vi "Base Level Estimation.vi"(7 "Base N info":T1, 8 "error in":errorcluster caption="エラー入力（エラーなし）", 9 "Filename":string, 10 "BR BL and STD info":T2, 11 "Raw data":dbl[](array[numeric])) -> (0 "error out":errorcluster caption="エラー出力", 2 "Data Estimated Info":T3, 3 "Relative G Data Array":dbl[](array[numeric]), 5 "Histogram Graph":T4(graph) caption="ヒストグラムグラフ")   [LabVIEW 2018]
uses:
  <vilib>/Analysis/baseanly.llb/Multimode.vi
  <vilib>/Analysis/baseanly.llb/Mean (DBL).vi
  <vilib>/Analysis/NI_AALBase.lvlib
panel:
  out "Region BL [pA]":dbl
  out "B BL [pA]":dbl
  out "H MIN Mode":dbl
  out "G level intensity":dbl
  out "要素":string
  out "Base S level":dbl[](array[numeric])
  out "Base Composition":string[](array[string])
  out "R Cut# 2":i32=15
  out "BL Level 2":dbl
  out "Mx Level intensity":dbl
  out "Mx level":dbl
  out "Histogram bin":dbl
  out "Data point":i32
  out "R Cut#":i32=15
  out "BL Level":dbl
  out "MIN":dbl
  out "MAX":dbl
  # "BL selection"
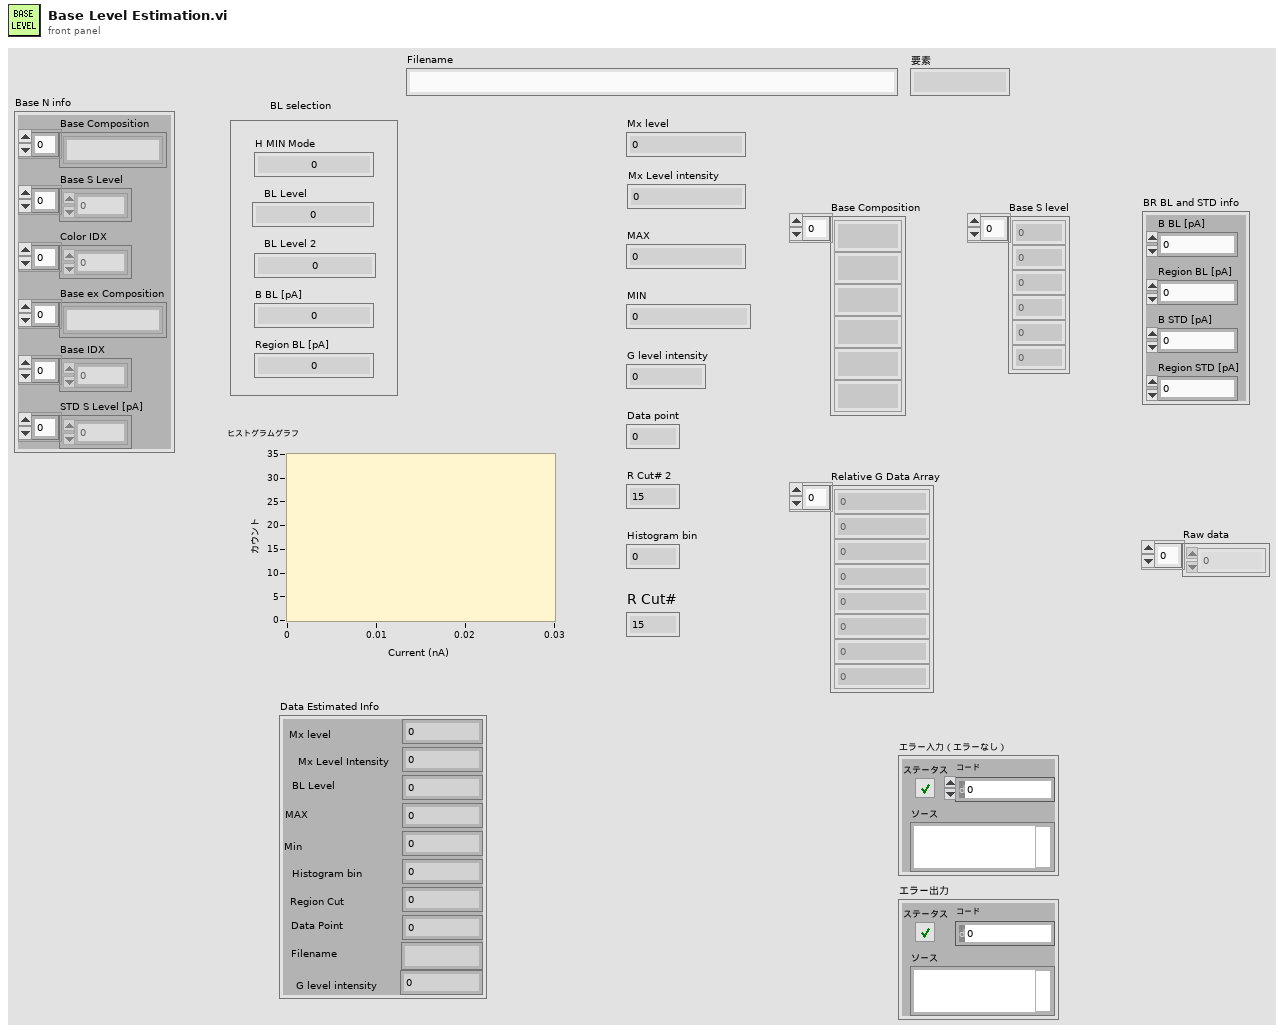
[diagram p1: front panel]
types:
  T1 = cluster{"Base Composition":string[], "Base S Level":dbl[], "Color IDX":u32[], "Base ex Composition":string[], "Base IDX":i32[], "STD S Level [pA]":dbl[]}
  T2 = cluster{"B BL [pA]":dbl, "Region BL [pA]":dbl, "B STD [pA]":dbl, "Region STD [pA]":dbl}
  T3 = cluster{"Mx level":dbl, "Mx Level Intensity":dbl, "BL Level":dbl, "MAX":dbl, "Min":dbl, "Histogram bin":dbl, "Region Cut":dbl, "Data Point":i32, "Filename":string, "G level intensity":dbl}
  T4 = cluster{"X Values":dbl[], "Histogram: h(x)":i32[]}
  T5 = cluster{dbl, dbl, dbl, dbl, dbl, "上限":dbl, dbl, i32, "Filename":string, dbl}
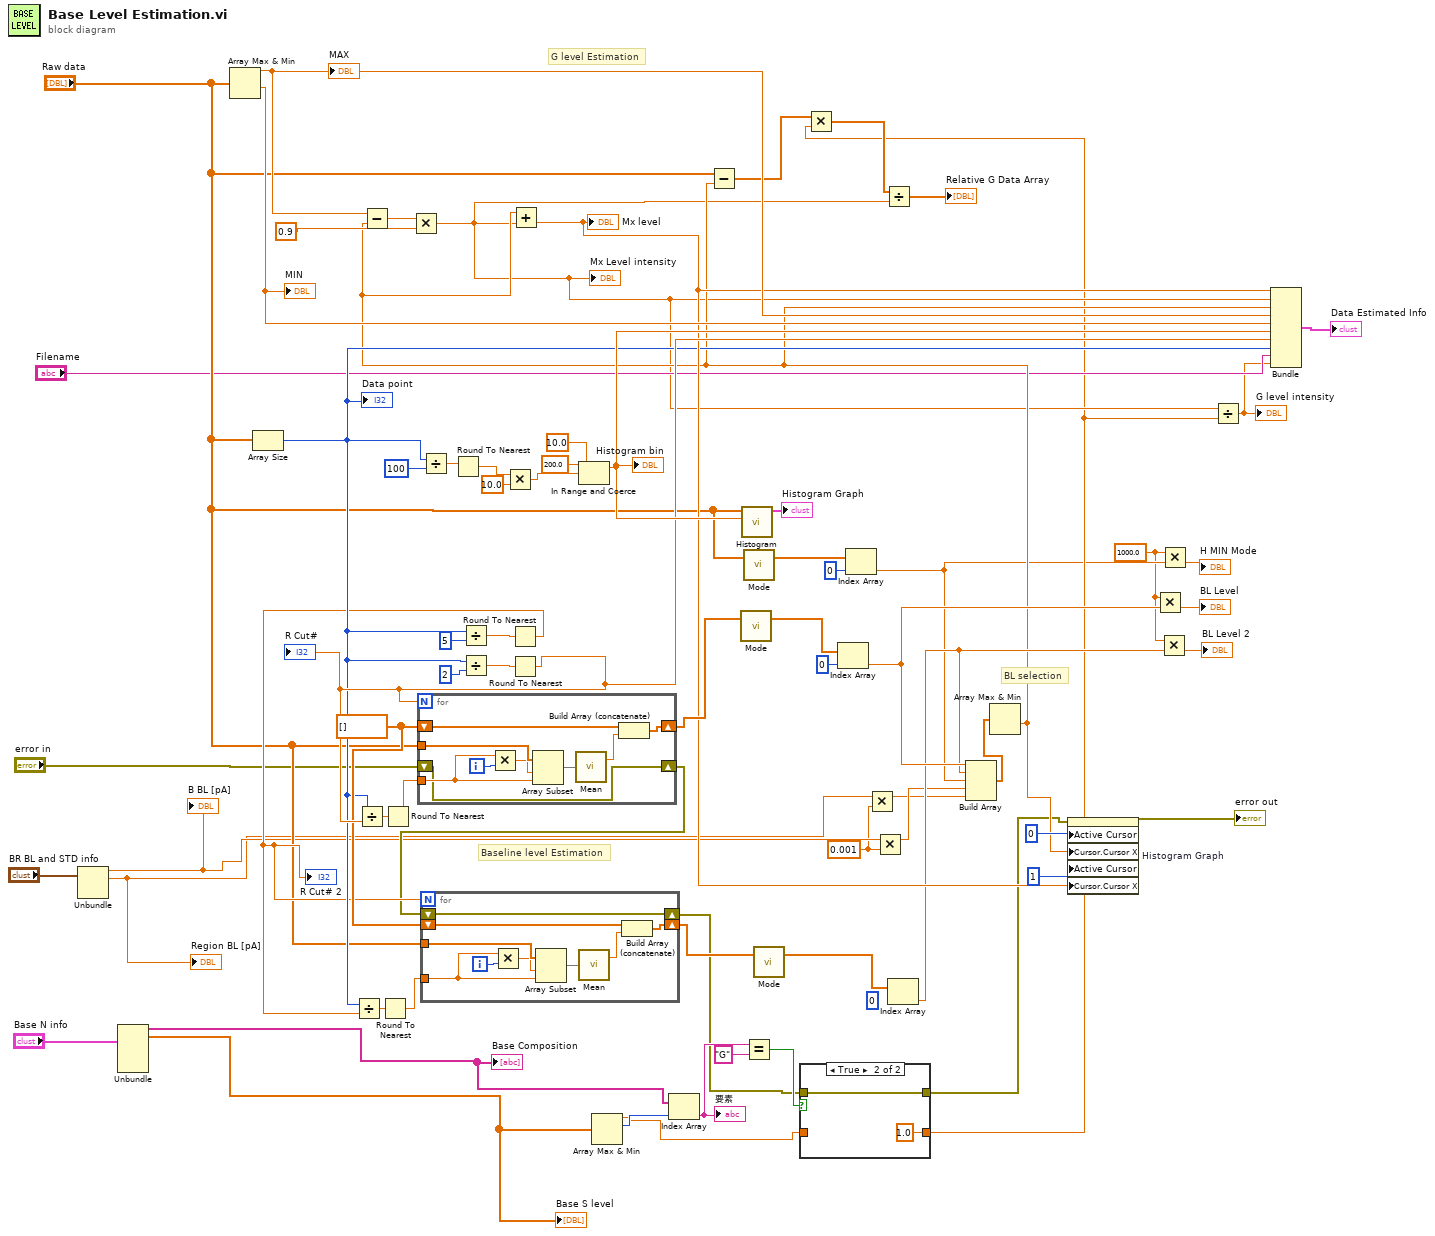
[diagram p0: block diagram]
diagram:
  w4 = 1000.0 ("x")
  w8 = 0.001 ("y")
  (unwired) 0 ("指標")
  w46 = dbl[] []
  # "BL selection"
  # "Baseline level Estimation"
  # "G level Estimation"
  n1 = Unbundle("BR BL and STD info") -> ("B BL [pA]"=w13:dbl, "Region BL [pA]"=w12:dbl)  [unwired: 2 out]
  "B BL [pA]" <- w13
  "Region BL [pA]" <- w12
  n2 = Unbundle("Base N info") -> ("Base Composition"=w2:string[], "Base S Level"=w1:dbl[])  [unwired: 4 out]
  "Base Composition" <- w2
  "Base S level" <- w1
  n3 = Array Max & Min(array="Raw data") -> (max value=w57:dbl, min value=w56:dbl)  [unwired: 2 out]
  "MAX" <- w57
  "MIN" <- w56
  n4 = Array Size(array="Raw data") -> (size(s)=w40:i32)
  "Data point" <- w40
  n5 = Divide(x=w40, y=100) -> (x/y=w69:dbl)
  n6 = Round To Nearest(number=w69) -> (nearest integer value=w68:dbl)
  n7 = Divide(x=w40, y=5) -> (x/y=w44:dbl)
  n8 = Divide(x=w40, y=2) -> (x/y=w59:dbl)
  n9 = Multiply(x=w68, y=10.0) -> (x*y=w66:dbl)
  n10 = Round To Nearest(number=w44) -> (nearest integer value=w39:dbl)
  "R Cut# 2" <- w39
  n11 = Divide(x=w40, y=w39) -> (x/y=w41:dbl)
  n12 = Round To Nearest(number=w41) -> (nearest integer value=w38:dbl)
  n13 = Round To Nearest(number=w59) -> (nearest integer value=w54:dbl)
  "R Cut#" <- w54
  n14 = Divide(x=w40, y=w54) -> (x/y=w72:dbl)
  n15 = Round To Nearest(number=w72) -> (nearest integer value=w58:dbl)
  n16 = for {
    N: w54 -> [_]
    tunnel: "Raw data" -> [w81]
    tunnel: w58 -> [w80]
    shift-right: [w75] -> w51
    shift-left: w46 -> [w74]
    shift-right: [w73] -> w20
    shift-left: "error in" -> [w73]
    i -> [w79]
    n17 = Multiply(x=w80, y=w79) -> (x*y=w78:dbl)
    n18 = Array Subset(array=w81, index=w78, length=w80) -> (w77:dbl[])
    n19 = call-poly <vilib>:"Mean.vi"("X"=w77) -> ("mean"=w76:dbl)  [unwired: 1 out]
    n20 = Build Array (concatenate)(w74, w76) -> (w75:dbl[])
  }
  n21 = for {
    N: w39 -> [_]
    tunnel: "Raw data" -> [w90]
    tunnel: w38 -> [w89]
    shift-right: [w84] -> w42
    shift-left: w46 -> [w83]
    shift-right: [w82] -> w19
    shift-left: w20 -> [w82]
    i -> [w88]
    n22 = Multiply(x=w89, y=w88) -> (x*y=w87:dbl)
    n23 = Array Subset(array=w90, index=w87, length=w89) -> (w86:dbl[])
    n24 = call-poly <vilib>:"Mean.vi"("X"=w86) -> ("mean"=w85:dbl)  [unwired: 1 out]
    n25 = Build Array (concatenate)(w83, w85) -> (w84:dbl[])
  }
  n26 = In Range and Coerce(upper limit=200.0 ("上限"), x=w66, lower limit=10.0 ("下限")) -> (coerced(x)=w55:dbl)  [unwired: 1 out]
  "Histogram bin" <- w55
  n27 = Array Max & Min(array=w1) -> (max value=w23:dbl, max index (indices)=w29:i32)  [unwired: 2 out]
  n28 = Index Array(array=w2, index=w29) -> (element=w26:string)
  "要素" <- w26
  n29 = call-poly <vilib>:"Mode.vi"("X"=w51) -> ("Modes"=w50:dbl[])  [unwired: 1 in, 1 out]
  n30 = call <vilib>:"Histogram.vi"("intervals"=w55, "X"="Raw data") -> ("Histogram Graph"=→"Histogram Graph":T4)  [unwired: 6 in, 3 out]
  n31 = call-poly <vilib>:"Mode.vi"("X"="Raw data") -> ("Modes"=w33:dbl[])  [unwired: 1 in, 1 out]
  n32 = Equal?(x=w26, y="G") -> (x = y?=w24:bool)
  n33 = call-poly <vilib>:"Mode.vi"("X"=w42) -> ("Modes"=w43:dbl[])  [unwired: 1 in, 1 out]
  n34 = case shown="True" w24 {
    tunnel: w23 -> [w92 _]
    tunnel: [w92 1.0] -> w16
    tunnel: w19 -> [w91 w93]
    tunnel: [w91 w93] -> w18
    frame False {
    }
    frame True {
    }
  }
  n35 = Index Array(array=w50, index=0 ("指標")) -> (element=w37:dbl)
  n36 = Index Array(array=w33, index=0 ("指標")) -> (element=w11:dbl)
  n37 = Multiply(x=w12, y=w8) -> (x*y=w9:dbl)
  n38 = Multiply(x=w13, y=w8) -> (x*y=w10:dbl)
  n39 = Index Array(array=w43) -> (element=w36:dbl)  [unwired: 1 in]
  n40 = Build Array(w37, w36, w11, w10, w9) -> (w35:dbl[])
  n41 = Array Max & Min(array=w35) -> (min value=w31:dbl)  [unwired: 3 out]
  n42 = Subtract(x=w57, y=w31) -> (x-y=w63:dbl)
  n43 = Multiply(x=w63, y=0.9) -> (x*y=w17:dbl)
  "Mx Level intensity" <- w17
  n44 = Add(x=w31, y=w17) -> (x+y=w47:dbl)
  "Mx level" <- w47
  n45 = Subtract(x="Raw data", y=w31) -> (x-y=w28:dbl[])
  n46 = Multiply(x=w28, y=w16) -> (x*y=w27:dbl[])
  n47 = Divide(x=w27, y=w17) -> (x/y=→"Relative G Data Array":dbl[])
  n48 = property on="Histogram Graph" class="XYGraph (strict)"(error in=w18, "Active Cursor"=u32 0 ("アクティブカーソル"), "Cursor.Cursor X"=w31, "Active Cursor"=u32 1 ("アクティブカーソル"), "Cursor.Cursor X"=w47) -> (error out=→"error out":errorcluster)  [unwired: 1 in, 1 out]
  n49 = Multiply(x=w4, y=w37) -> (x*y=→"BL Level":dbl)
  n50 = Multiply(x=w4, y=w36) -> (x*y=→"BL Level 2":dbl)
  n51 = Multiply(x=w4, y=w11) -> (x*y=→"H MIN Mode":dbl)
  n52 = Divide(x=w17, y=w16) -> (x/y=w15:dbl)
  "G level intensity" <- w15
  n53 = Bundle(w47, w17, w31, w57, w56, "上限"=w55, w54, w40, "Filename"="Filename", w15) -> (→"Data Estimated Info":T5)  [unwired: 1 in]
